vi "Own20261012_SetPropertyItem.vi"() -> ()   [LabVIEW 2024]
panel:
  out "error out":errorcluster caption="错误输出"
  in  "allow_alternate_names":bool
  in  "property_id_string":string
  in  "property_item_id":u32
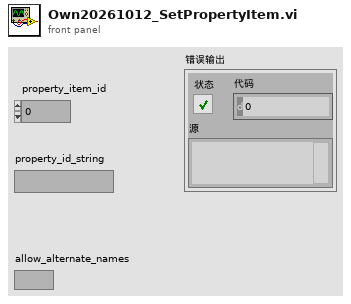
[diagram p1: front panel]
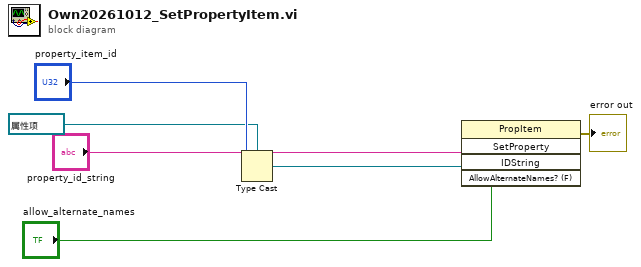
[diagram p0: block diagram]
diagram:
  n1 = Type Cast(type=refnum<vi> refnum ("引用"), x="property_item_id") -> (*(type *) &x=w4:refnum<vi>)
  n2 = invoke class="PropItem" method="SetProperty"(reference=w4, "IDString"="property_id_string", "AllowAlternateNames? (F)"="allow_alternate_names") -> (error out=→"error out":errorcluster)  [unwired: 2 in, 4 out]
